vi "Read Macro Steps.vi"(8 "error in (no error)":errorcluster, 10 "Schema Version":string, 11 "refnum":T3) -> (0 "error out":errorcluster, 2 "Macro Steps":T1[](array[typedef]), 3 "refnum out":T3)   [LabVIEW 2023]
doc: "Reads the list of steps from macro config file defined by <B>refnum</B>."
uses:
  <vilib>/Utility/config.llb/Config Data RefNum.ctl
  CTLs/Step V3.ctl
  CTLs/Step Type V3.ctl
  <vilib>/Utility/config.llb/Read Key (I32).vi
  <vilib>/Utility/config.llb/Read Key (String).vi
  <vilib>/Utility/error.llb/Error Cluster From Error Code.vi
  <vilib>/ErrorRing/Error Ring.xnode
  <vilib>/Utility/config.llb/Read Key (U32).vi
  <vilib>/Utility/config.llb/Read Key (Boolean).vi
  <vilib>/Utility/config.llb/NI_LVConfig.lvlib
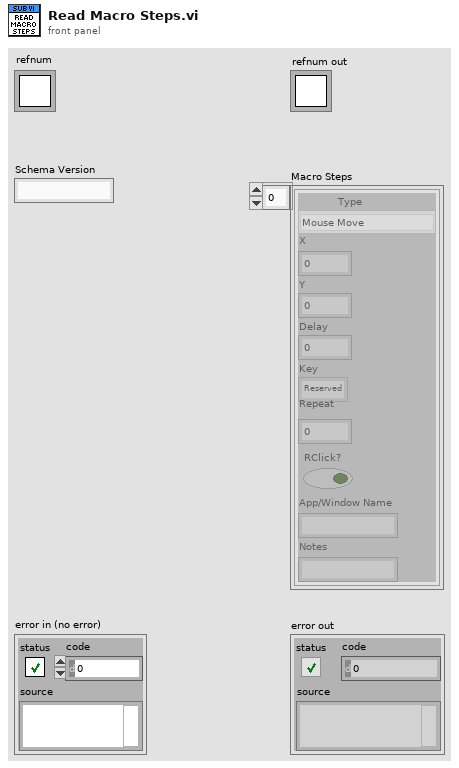
[diagram p1: front panel]
types:
  T1 = typedef "Step V3.ctl" = cluster{"Type":T2, "X":i32, "Y":i32, "Delay":i32, "Key":u8, "Repeat":i32, "RClick?":bool, "App/Window Name":string, "Notes":string}
  T2 = typedef "Step Type V3.ctl" = enum16{"Mouse Move", "Mouse Click", "Key Press", "Wait", "Mouse Down", "Mouse Up", "Key Down", "Key Up", "Run Application", "Maximize Window", "Restore Window", "Minimize Window", "Close Window", "Bring Window to Front", "Send Window to Back"}
  T3 = typedef "NI_LVConfig.lvlib/Config Data RefNum.ctl" = refnum<k1>
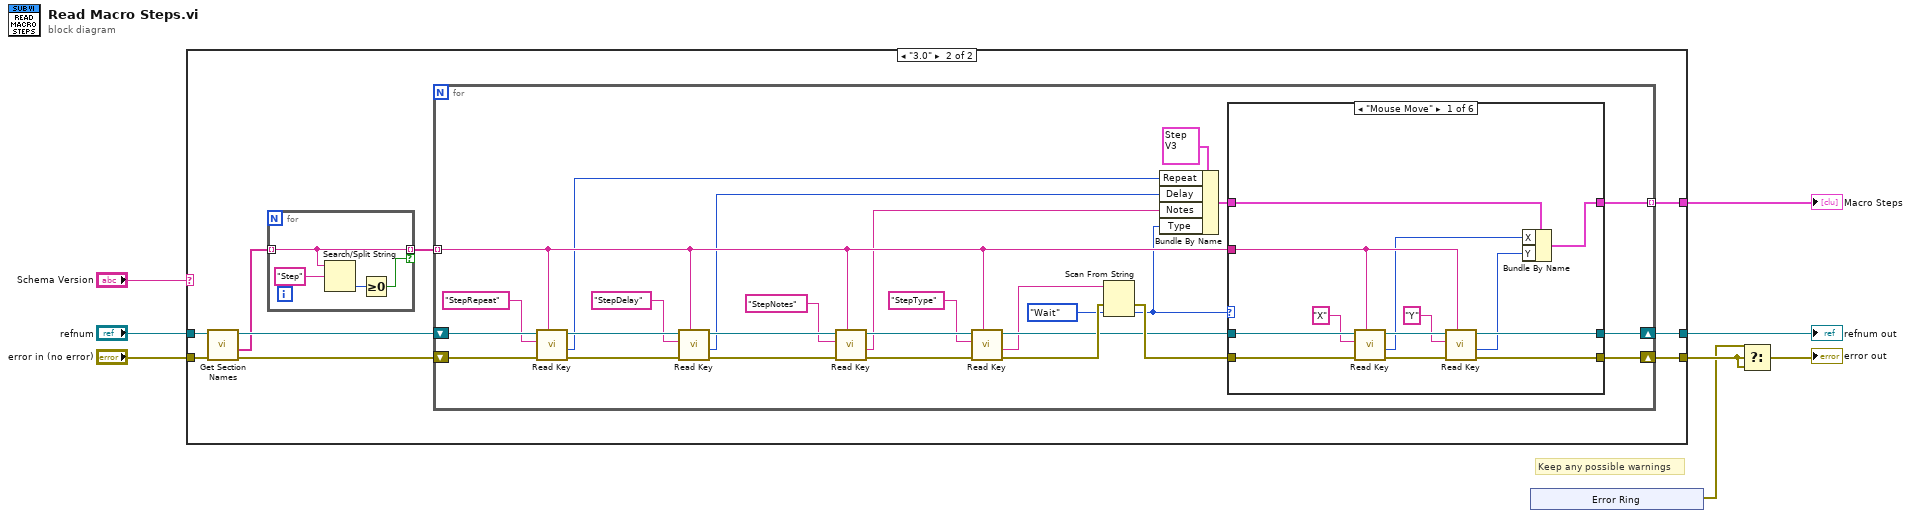
[diagram p0: block diagram]
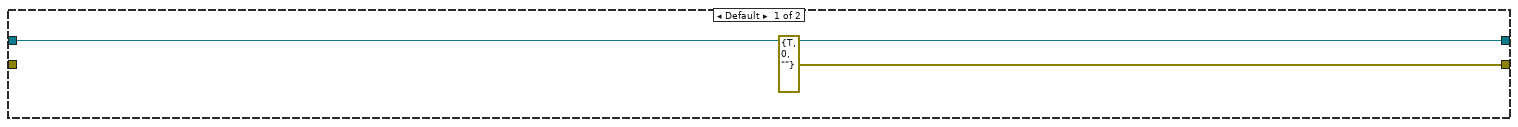
[diagram p2: hidden frame]
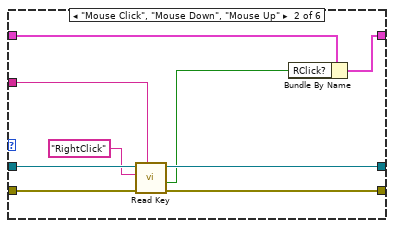
[diagram p3: hidden frame]
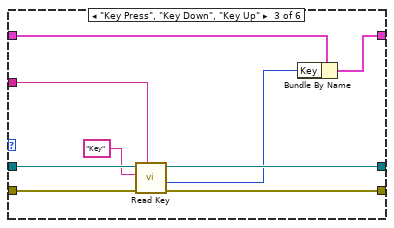
[diagram p4: hidden frame]
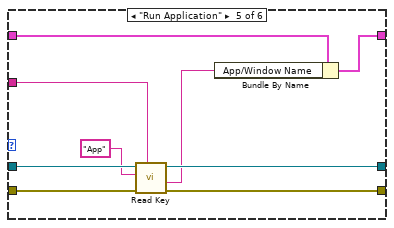
[diagram p6: hidden frame]
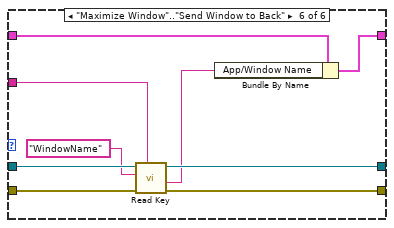
[diagram p7: hidden frame]
diagram:
  # "Keep any possible warnings"
  n1 = case shown="\"3.0\"" "Schema Version" {
    tunnel: "refnum" -> [w10 w16]
    tunnel: [w10 w18] -> w2
    tunnel: [errorcluster {"status"=TRUE, "code"=0, "source"=""} ("error out") w19] -> w8
    tunnel: "error in (no error)" -> [_ w17]
    tunnel: [_ w12] -> w1
    frame Default {
    }
    frame "3.0" {
      n2 = call <vilib>:"Get Section Names.vi"("error in (no error)"=w17, "refnum"=w16) -> ("error out"=w15:errorcluster, "section names"=w13:string[], "refnum out"=w14:T3)  [unwired: 7 in]
      n3 = for {
        tunnel: w13 -> [w99] mode=indexing
        tunnel: [w99] -> w11 mode=indexing if=w100
        n4 = Search/Split String(string=w99, search string/char (-)="Step") -> (offset of match=w101:i32)  [unwired: 1 in, 2 out]
        n5 = Greater Or Equal To 0?(x=w101) -> (x >= 0?=w100:bool)
      }
      n6 = for {
        tunnel: [w35] -> w12 mode=indexing
        shift-right: [w37] -> w19
        shift-left: w15 -> [w40]
        shift-right: [w36] -> w18
        shift-left: w14 -> [w41]
        tunnel: w11 -> [w26] mode=indexing
        n7 = call-poly <vilib>:"Read Key.vi"("section"=w26, "error in (no error)"=w40, "key"="StepRepeat", "refnum"=w41) -> ("error out"=w32:errorcluster, "value"=w24:i32, "refnum out"=w42:T3)  [unwired: 4 in, 1 out]
        n8 = call-poly <vilib>:"Read Key.vi"("section"=w26, "error in (no error)"=w32, "key"="StepDelay", "refnum"=w42) -> ("error out"=w31:errorcluster, "value"=w23:i32, "refnum out"=w44:T3)  [unwired: 4 in, 1 out]
        n9 = call-poly <vilib>:"Read Key.vi"("section"=w26, "error in (no error)"=w31, "key"="StepNotes" ("section"), "refnum"=w44) -> ("error out"=w28:errorcluster, "value"=w22:string, "refnum out"=w43:T3)  [unwired: 4 in, 1 out]
        n10 = call-poly <vilib>:"Read Key.vi"("section"=w26, "error in (no error)"=w28, "key"="StepType", "refnum"=w43) -> ("error out"=w45:errorcluster, "value"=w29:string, "refnum out"=w30:T3)  [unwired: 4 in, 1 out]
        n11 = Scan From String(input string=w29, error in=w45, default 1=Step_Type_V3."Wait" ("Step Type")) -> (error out=w46:errorcluster, output 1=w21:T2)  [unwired: 2 in, 2 out]
        n12 = Bundle By Name(cluster=T1 {"Type"=enum."Mouse Move", "X"=0, "Y"=0, "Delay"=0, "Key"=65, "Repeat"=0, "RClick?"=FALSE, "App/Window Name"="", "Notes"=""} ("Step"), "Repeat"=w24, "Delay"=w23, "Notes"=w22, "Type"=w21) -> (w20:T1)
        n13 = case shown="\"Mouse Move\"" w21 {
          tunnel: w46 -> [w58 w68 w77 w79 w89 w98]
          tunnel: w30 -> [w57 w67 w76 w80 w88 w97]
          tunnel: w26 -> [w53 w65 w74 _ w86 w95]
          tunnel: [w52 w62 w71 w79 w83 w92] -> w37
          tunnel: [w51 w64 w72 w80 w84 w93] -> w36
          tunnel: [w48 w60 w73 w78 w85 w94] -> w35
          tunnel: w20 -> [w47 w61 w69 w78 w81 w90]
          frame "Mouse Move" {
            n14 = call-poly <vilib>:"Read Key.vi"("section"=w53, "error in (no error)"=w58, "key"="X", "refnum"=w57) -> ("error out"=w54:errorcluster, "value"=w50:i32, "refnum out"=w59:T3)  [unwired: 4 in, 1 out]
            n15 = call-poly <vilib>:"Read Key.vi"("section"=w53, "error in (no error)"=w54, "key"="Y", "refnum"=w59) -> ("error out"=w52:errorcluster, "value"=w49:i32, "refnum out"=w51:T3)  [unwired: 4 in, 1 out]
            n16 = Bundle By Name(cluster=w47, "X"=w50, "Y"=w49) -> (w48:T1)
          }
          frame "Mouse Click", "Mouse Down", "Mouse Up" {
            n17 = call-poly <vilib>:"Read Key.vi"("section"=w65, "error in (no error)"=w68, "key"="RightClick", "refnum"=w67) -> ("error out"=w62:errorcluster, "value"=w63:bool, "refnum out"=w64:T3)  [unwired: 4 in, 1 out]
            n18 = Bundle By Name(cluster=w61, "RClick?"=w63) -> (w60:T1)
          }
          frame "Key Press", "Key Down", "Key Up" {
            n19 = call-poly <vilib>:"Read Key.vi"("section"=w74, "error in (no error)"=w77, "key"="Key", "refnum"=w76) -> ("error out"=w71:errorcluster, "value"=w70:u32, "refnum out"=w72:T3)  [unwired: 4 in, 1 out]
            n20 = Bundle By Name(cluster=w69, "Key"=w70) -> (w73:T1)
          }
          frame "Wait" {
          }
          frame "Run Application" {
            n21 = call-poly <vilib>:"Read Key.vi"("section"=w86, "error in (no error)"=w89, "key"="App", "refnum"=w88) -> ("error out"=w83:errorcluster, "value"=w82:string, "refnum out"=w84:T3)  [unwired: 4 in, 1 out]
            n22 = Bundle By Name(cluster=w81, "App/Window Name"=w82) -> (w85:T1)
          }
          frame "Maximize Window".."Send Window to Back" {
            n23 = call-poly <vilib>:"Read Key.vi"("section"=w95, "error in (no error)"=w98, "key"="WindowName", "refnum"=w97) -> ("error out"=w92:errorcluster, "value"=w91:string, "refnum out"=w93:T3)  [unwired: 4 in, 1 out]
            n24 = Bundle By Name(cluster=w90, "App/Window Name"=w91) -> (w94:T1)
          }
        }
      }
    }
  }
  "refnum out" <- w2
  "Macro Steps" <- w1
  n25 = xnode "Error Ring"() -> ("error out"=w7:errorcluster)
  n26 = Select(t=w7, s=w8, f=w8) -> (s? t:f=→"error out":errorcluster)
